vi "Generate Packet Identifier.vi"() -> (2 "Packet Identifier":u16 format="%04x")   [LabVIEW 2013, in "MQTT_Control_Packets.lvlib" / "ControlPacket.lvclass"]
uses:
  ControlPacket.lvclass
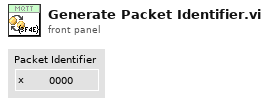
[diagram p1: front panel]
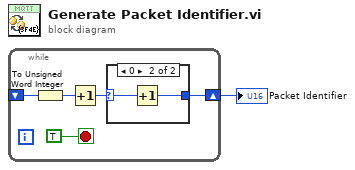
[diagram p0: block diagram]
diagram:
  n1 = while {
    shift-right: [w3] -> w1
    shift-left: _ -> [w5]
    stop <- TRUE stop-if-true
    n2 = To Unsigned Word Integer(number=w5) -> (unsigned 16bit integer=w4:u16)
    n3 = Increment(x=w4) -> (x+1=w2:u16)
    n4 = case shown="0" w2 {
      selector: w2 -> [w7 w8]
      tunnel: [w7 w9] -> w3
      frame Default {
      }
      frame 0 {
        n5 = Increment(x=w8) -> (x+1=w9:u16)
      }
    }
  }
  "Packet Identifier" <- w1
